vi "Determine If Belongs In Sector and Accumulate.vi"(6 "Left Sector Parameters":T3, 7 "Right Sector Parameters":T3, 8 "error in (no error)":errorcluster, 9 "Midpoint of Image":dbl, 10 "Starting Y Location":i32, 11 "Image Data":u8[][](array[numeric])) -> (0 "error out":errorcluster, 2 "Canceled?":bool, 3 "[Accumulated Sectors]":T2[](array[typedef]))   [LabVIEW 2013]
uses:
  FPGA/Sector/Accumulate/Sector Parameter Cluster.ctl
  FPGA/Sector/Accumulate/Accumulated Sector Cluster.ctl
  Test Compiliation/Test Sector Cluster.ctl
  FPGA/FPGA Image Processing.lvlib
panel:
  out "Pixel Sectors":T1[](array[typedef])
  in  "Cancel Button":bool
  out "Progress":u16(slide) scale=0.0..788.0
  # "Calculating Average Sector Background ..."
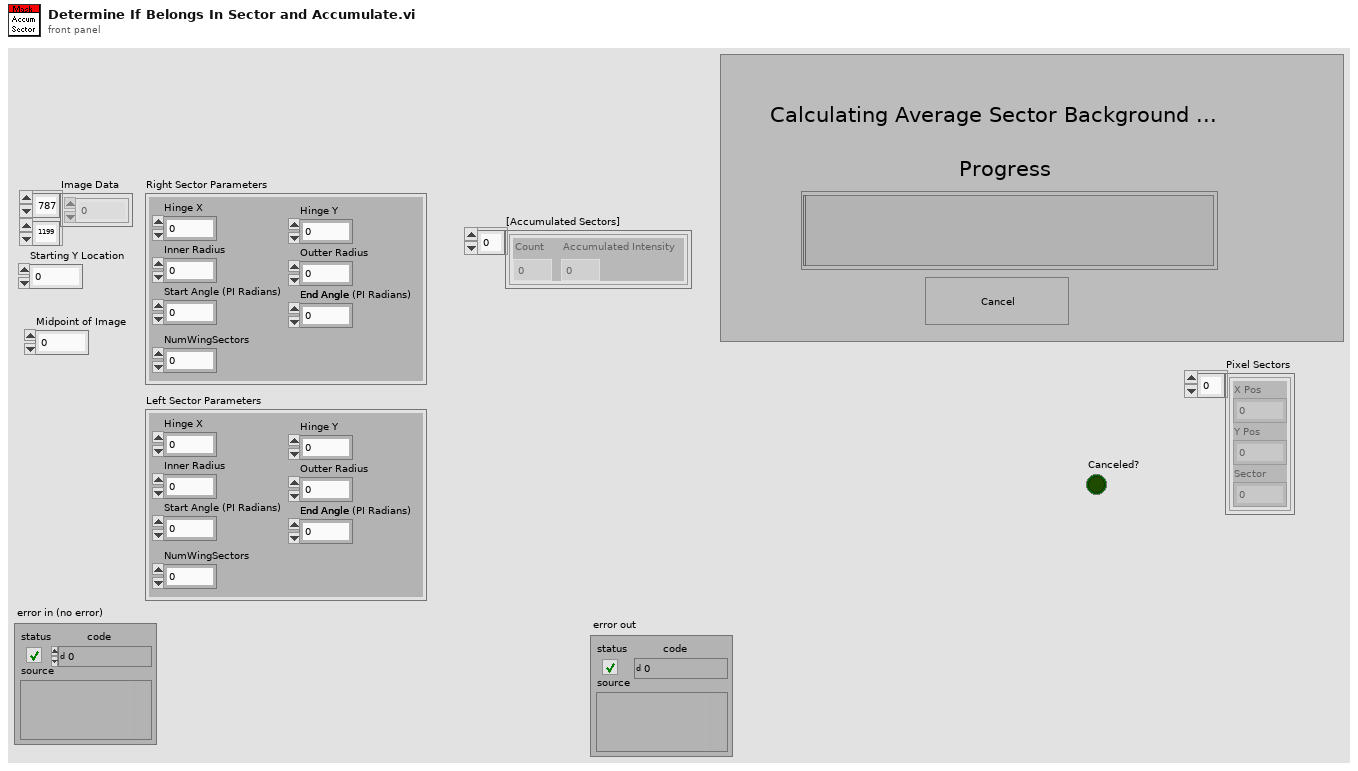
[diagram p1: front panel]
types:
  T1 = typedef "Test Sector Cluster.ctl" = cluster{"X Pos":u16, "Y Pos":u16, "Sector":u8}
  T2 = typedef "Accumulated Sector Cluster.ctl" = cluster{"Accumulated Intensity":u32, "Count":u16}
  T3 = typedef "Sector Parameter Cluster.ctl" = cluster{"Start Angle":fxp<+/-,17,2>, "End Angle":fxp<+,17,3>, "Inner Radius":u16, "Outter Radius":u16, "Hinge X":u16, "Hinge Y":u16, "NumWingSectors":u8}
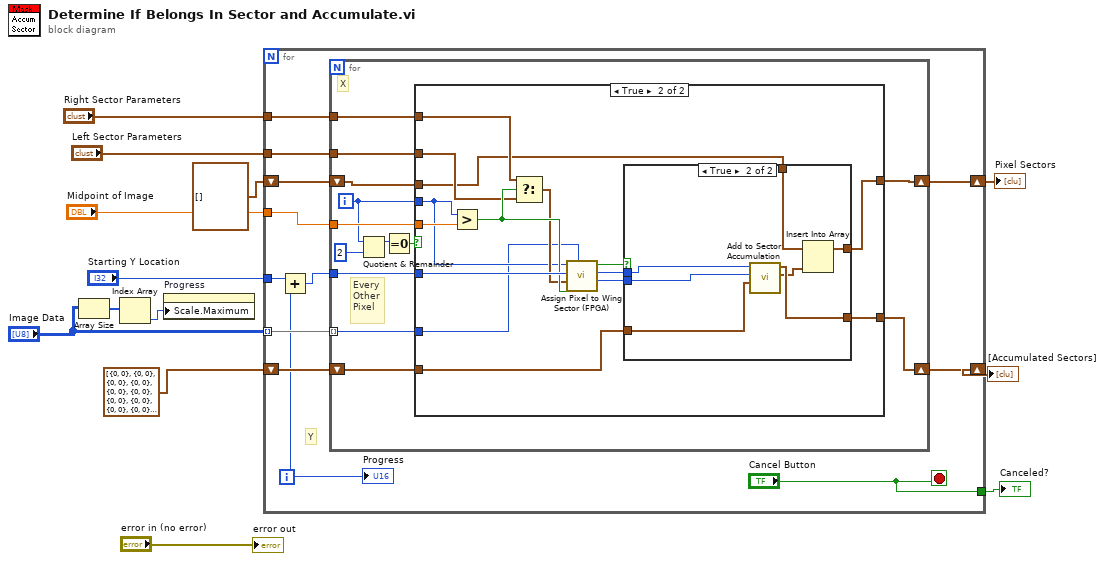
[diagram p0: block diagram]
diagram:
  n1 = Array Size(array="Image Data") -> (size(s)=w5:i32[])
  n2 = Index Array(array=w5) -> (element=w4:i32)  [unwired: 1 in]
  n3 = property on="Progress" class="Slide (strict)"("Scale.Maximum"=w4) -> ()  [unwired: 2 in, 2 out]
  n4 = for {
    tunnel: "Image Data" -> [w25] mode=indexing
    tunnel: "Midpoint of Image" -> [w24]
    tunnel: "Right Sector Parameters" -> [w23]
    tunnel: "Left Sector Parameters" -> [w22]
    shift-right: [w20] -> w8
    shift-left: T2[] [{"Accumulated Intensity"=0, "Count"=0}, {"Accumulated Intensity"=0, "Count"=0}, {"Accumulated Intensity"=0, "Count"=0}, {"Accumulated Intensity"=0, "Count"=0}, {"Accumulated Intensity"=0, "Count"=0}, {"Accumulated Intensity"=0, "Count"=0}, {"Accumulated Intensity"=0, "Count"=0}, {"Accumulated Intensity"=0, "Count"=0}, {"Accumulated Intensity"=0, "Count"=0}, {"Accumulated Intensity"=0, "Count"=0}, {"Accumulated Intensity"=0, "Count"=0}, {"Accumulated Intensity"=0, "Count"=0}, {"Accumulated Intensity"=0, "Count"=0}, {"Accumulated Intensity"=0, "Count"=0}, {"Accumulated Intensity"=0, "Count"=0}, {"Accumulated Intensity"=0, "Count"=0}, {"Accumulated Intensity"=0, "Count"=0}, {"Accumulated Intensity"=0, "Count"=0}, {"Accumulated Intensity"=0, "Count"=0}, {"Accumulated Intensity"=0, "Count"=0}, {"Accumulated Intensity"=0, "Count"=0}, {"Accumulated Intensity"=0, "Count"=0}, {"Accumulated Intensity"=0, "Count"=0}, {"Accumulated Intensity"=0, "Count"=0}, {"Accumulated Intensity"=0, "Count"=0}, {"Accumulated Intensity"=0, "Count"=0}, {"Accumulated Intensity"=0, "Count"=0}, {"Accumulated Intensity"=0, "Count"=0}, {"Accumulated Intensity"=0, "Count"=0}, {"Accumulated Intensity"=0, "Count"=0}, {"Accumulated Intensity"=0, "Count"=0}, {"Accumulated Intensity"=0, "Count"=0}] ("[Accumulated Sectors] Out") -> [w21]
    tunnel: "Starting Y Location" -> [w18]
    tunnel: ["Cancel Button"] -> w3
    shift-right: [w14] -> w1
    shift-left: T1[] [] ("array") -> [w15]
    i -> [w17]
    stop <- "Cancel Button" stop-if-true
    # "Y"
    n5 = Add(x=w18, y=w17) -> (x+y=w19:i32)
    n6 = for {
      tunnel: w25 -> [w34] mode=indexing
      tunnel: w19 -> [w38]
      tunnel: w24 -> [w37]
      tunnel: w23 -> [w36]
      tunnel: w22 -> [w35]
      shift-right: [w32] -> w20
      shift-left: w21 -> [w33]
      shift-right: [w26] -> w14
      shift-left: w15 -> [w27]
      i -> [w31]
      # "Every\nOther\nPixel"
      # "X"
      n7 = Quotient & Remainder(x=w31, y=2) -> (x-y*floor(x/y)=w29:i32)  [unwired: 1 out]
      n8 = Equal To 0?(x=w29) -> (x = 0?=w28:bool)
      n9 = case shown="True" w28 {
        tunnel: w38 -> [_ w55]
        tunnel: w37 -> [_ w54]
        tunnel: w36 -> [_ w52]
        tunnel: w35 -> [_ w51]
        tunnel: w31 -> [_ w49]
        tunnel: w34 -> [_ w48]
        tunnel: w33 -> [w40 w46]
        tunnel: [w40 w44] -> w32
        tunnel: w27 -> [w39 w42]
        tunnel: [w39 w41] -> w26
        frame False {
        }
        frame True {
          n10 = Greater?(x=w49, y=w54) -> (0:w53:bool)
          n11 = Select(t=w52, s=w53, f=w51) -> (s? t:f=w50:T3)
          n12 = call "Assign Pixel to Wing Sector (FPGA).vi"("Pixel Intensity In"=w48, "Right Wing?"=w53, "Sector Parameters"=w50, "Pixel Y"=w55, "Pixel X"=w49) -> ("Pixel Intensity Out"=w43:u8, "sector #"=w45:u8, "output valid"=w47:bool)  [unwired: 3 in]
          n13 = case shown="True" w47 {
            tunnel: w46 -> [w57 w62]
            tunnel: w45 -> [_ w64]
            tunnel: [w57 w61] -> w44
            tunnel: w43 -> [_ w63]
            tunnel: w42 -> [w56 w58]
            tunnel: [w56 w60] -> w41
            frame False {
            }
            frame True {
              n14 = call "Add to Sector Accumulation.vi"("[Accumulated Sectors] In"=w62, "Pixel Intensity"=w63, "Sector ID"=w64) -> ("Sector Pixel"=w59:T1, "[Accumulated Sectors] Out"=w61:T2[])  [unwired: 7 in]
              n15 = Insert Into Array(array=w58, new element=w59) -> (w60:T1[])  [unwired: 1 in]
            }
          }
        }
      }
    }
    "Progress" <- w17
  }
  "[Accumulated Sectors]" <- w8
  "Canceled?" <- w3
  "Pixel Sectors" <- w1
  "error out" <- "error in (no error)"
